vi "Connect.vi"(8 "error in (no error)":errorcluster caption="에러 입력(에러 없음)", 9 "원격 포트 또는 서비스 이름":u16, 10 "주소":string, 11 "CE RF Switch Box 입력":refnum<class "CE RF Switch Box.lvclass">) -> (0 "error out":errorcluster caption="에러 출력", 2 "Connected?":bool, 3 "CE RF Switch Box 출력":refnum<class "CE RF Switch Box.lvclass">)   [LabVIEW 2023, in "RF Switch Box.lvlib" / "CE RF Switch Box.lvclass"]
uses:
  CE RF Switch Box.lvclass
  CE RF Switch Box.lvclass/CE RF Switch Box.ctl
panel:
  out "데이터 출력":string
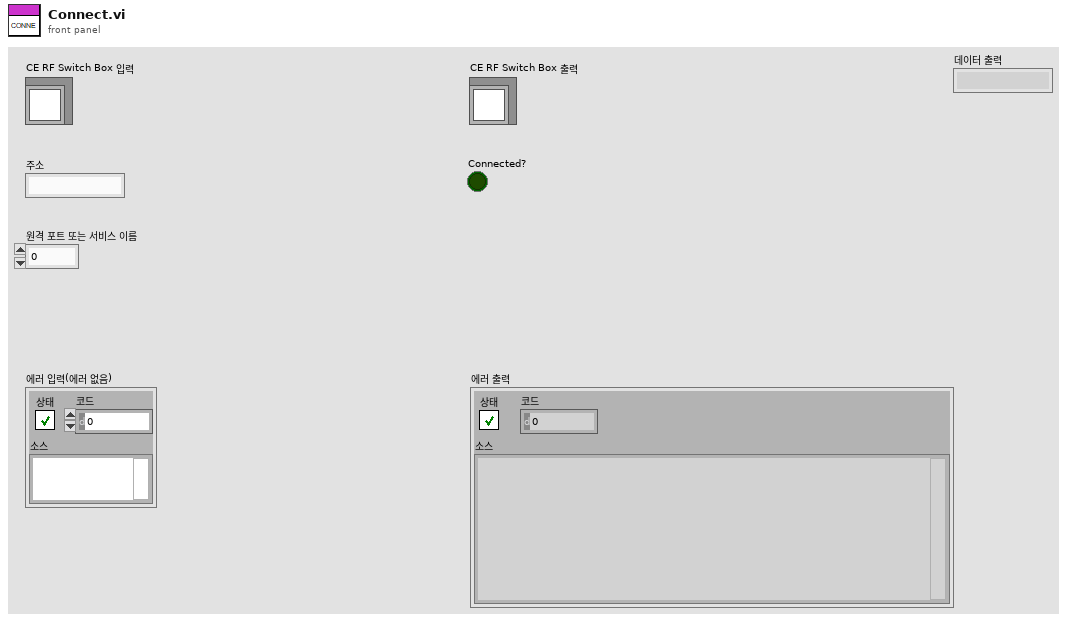
[diagram p1: front panel]
types:
  T1 = enum16{"Standard", "Buffered", "CRLF", "Immediate"}
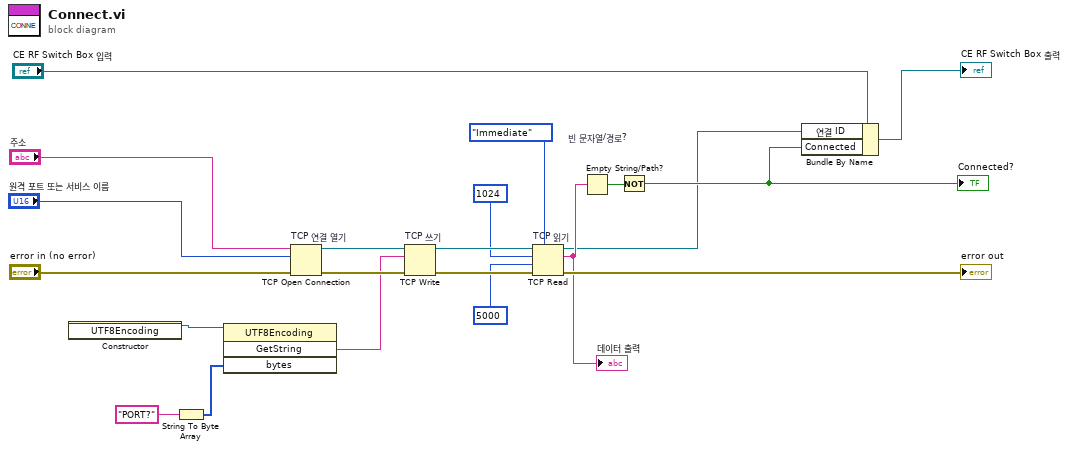
[diagram p0: block diagram]
diagram:
  n1 = constructor class="UTF8Encoding"() -> (reference out=w8:refnum<k24>)  [unwired: 3 in, 2 out]
  n2 = String To Byte Array(string="PORT?" ("데이터 입력")) -> (unsigned byte array=w5:u8[])
  n3 = invoke class="UTF8Encoding" method="GetString"(reference=w8, "bytes"=w5) -> ("GetString"=w6:string)  [unwired: 2 in, 3 out]
  n4 = TCP Open Connection "TCP 연결 열기"(address="주소", remote port or service name="원격 포트 또는 서비스 이름", error in (no error)="error in (no error)") -> (connection ID=w18:refnum<k5>, error out=w17:errorcluster)  [unwired: 2 in]
  n5 = TCP Write "TCP 쓰기"(connection ID=w18, data in=w6, error in (no error)=w17) -> (connection ID out=w15:refnum<k5>, error out=w16:errorcluster)  [unwired: 1 in, 1 out]
  n6 = TCP Read "TCP 읽기"(connection ID=w15, bytes to read=1024 ("읽을 바이트"), error in (no error)=w16, 7:T1."Immediate" ("모드(standard)"), 9:5000 ("타임아웃 ms (25000)")) -> (connection ID out=w1:refnum<k5>, data out=w3:string, error out=→"error out":errorcluster)
  "데이터 출력" <- w3
  n7 = Empty String/Path? "빈 문자열/경로?"(string/path=w3) -> (empty?=w13:bool)
  n8 = Not(x=w13) -> (.not. x?=w9:bool)
  "Connected?" <- w9
  n9 = Bundle By Name(cluster="CE RF Switch Box 입력", "연결 ID"=w1, "Connected"=w9) -> (→"CE RF Switch Box 출력":refnum<class "CE RF Switch Box.lvclass">)
